vi "Check Trigger Conditions.vi"(7 "Force Trigger?":bool, 8 "error in (no error)":errorcluster, 9 "Waveform Data":waveform(sgl)[](array[waveform]), 10 "Acquisition and Logging Configuration":T1={"Data Rate"=1, "Samples per Read"=0, "Number of Reads to Save"=0, "Data File Name"="", "TDMS Properties"=[], "Number of Channels"=4, "Channel Scale Array"=[0.0, 0.0, 0.0, 0.0, 1.0, 1.0, 1.0, 1.0, 1.0, 1.0, 1.0, 1.0, 1.0, 1.0, 1.0, 1.0], "Channel Names"=[], "Trigger - RMS Value"=0.0, "Trigger - Channel"=0, "Trigger - Time (Minute)"=0, "Frequency "=0, "Amplitude (0~10)"=0.0} {"Amplitude (0~10)" min=-10.0 max=10.0; "Data Rate" items=["50.000 kS/s (NI 9239)"=1, "25.000 kS/s (NI 9239)"=2, "16.667 kS/s (NI 9239)"=3, "12.500 kS/s (NI 9239)"=4, "10.000 kS/s (NI 9239)"=5, "8.333 kS/s (NI 9239)"=6, "7.143 kS/s (NI 9239)"=7, "6.250 kS/s (NI 9239)"=8, "5.556 kS/s (NI 9239)"=9, "5.000 kS/s (NI 9239)"=10, "4.545 kS/s (NI 9239)"=11, "4.167 kS/s (NI 9239)"=12, "3.846 kS/s (NI 9239)"=13, "3.571 kS/s (NI 9239)"=14, "3.333 kS/s (NI 9239)"=15, "3.125 kS/s (NI 9239)"=16, "2.941 kS/s (NI 9239)"=17, "2.778 kS/s (NI 9239)"=18, "2.632 kS/s (NI 9239)"=19, "2.500 kS/s (NI 9239)"=20, "2.381 kS/s (NI 9239)"=21, "2.273 kS/s (NI 9239)"=22, "2.174 kS/s (NI 9239)"=23, "2.083 kS/s (NI 9239)"=24, "2.000 kS/s (NI 9239)"=25, "1.923 kS/s (NI 9239)"=26, "1.852 kS/s (NI 9239)"=27, "1.786 kS/s (NI 9239)"=28, "1.724 kS/s (NI 9239)"=29, "1.667 kS/s (NI 9239)"=30, "1.613 kS/s (NI 9239)"=31]}) -> (0 "error out":errorcluster, 3 "Trigger Condition Met?":bool)   [LabVIEW 2016]
uses:
  controls/Acquisition and Logging Configuration.ctl
  <vilib>/LabVIEW Targets/FPGA/cRIO/shared/nicrio_ModuleControls/nicrio_cRIO-9239_DataRatesRing.ctl
  controls/TDMS Properties.ctl
  <vilib>/Analysis/5stat.llb/RMS (DBL).vi
  <vilib>/Analysis/NI_AALPro.lvlib
panel:
  # "Verifica condições para início da aquisição, são elas:\n• Caso trigger seja forçado pela usuário\n• Caso o contador chegue no múltiplo correspondente ao Trigger - Time(Minute)\n• Caso o valor da forma de onda no canal escolhido seja alcançado\n• No caso do Trigger Minute = 0, dentro do arquivo de configuração, \nfoi convencionado que esse trigger sempre estará acionado para que aquisição nunca termine.\nEssa funcionalidade está documentada no diagrama de blocos."
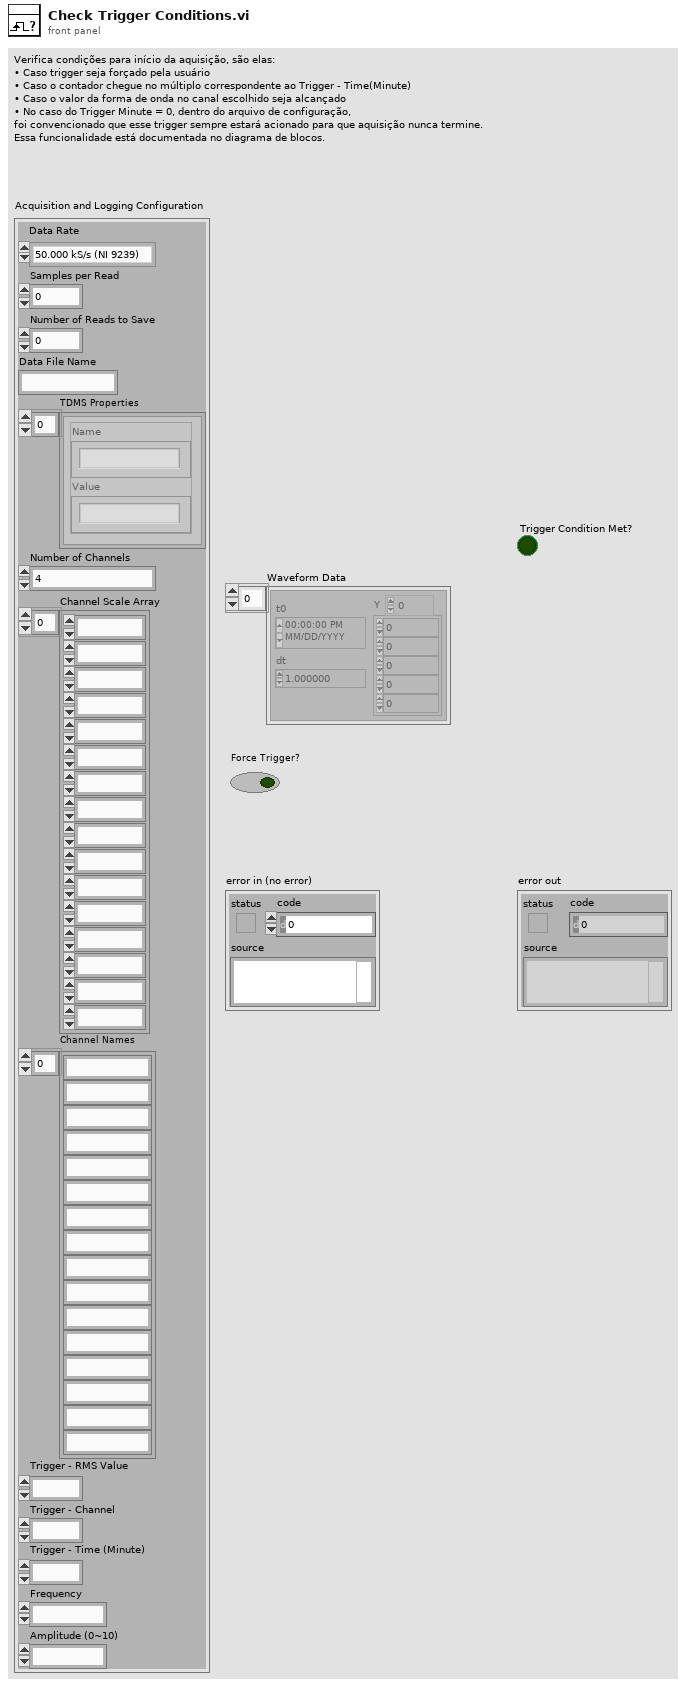
[diagram p1: front panel]
types:
  T1 = typedef "Acquisition and Logging Configuration.ctl" = cluster{"Data Rate":T2, "Samples per Read":i32, "Number of Reads to Save":i32, "Data File Name":string, "TDMS Properties":T3[], "Number of Channels":i32, "Channel Scale Array":fxp<+,24,12>[], "Channel Names":string[], "Trigger - RMS Value":dbl, "Trigger - Channel":i32, "Trigger - Time (Minute)":i32, "Frequency ":i32, "Amplitude (0~10)":dbl}
  T2 = typedef "nicrio_cRIO-9239_DataRatesRing.ctl" = u8
  T3 = typedef "TDMS Properties.ctl" = cluster{"Name":string, "Value":string}
  T4 = typedef "LVDateTimeRec.ctl" = cluster{"fractional second":dbl, "second":i32, "minute":i32, "hour":i32, "day of month":i32, "month":i32, "year":i32, "day of week":i32, "day of year":i32, "DST":i32}
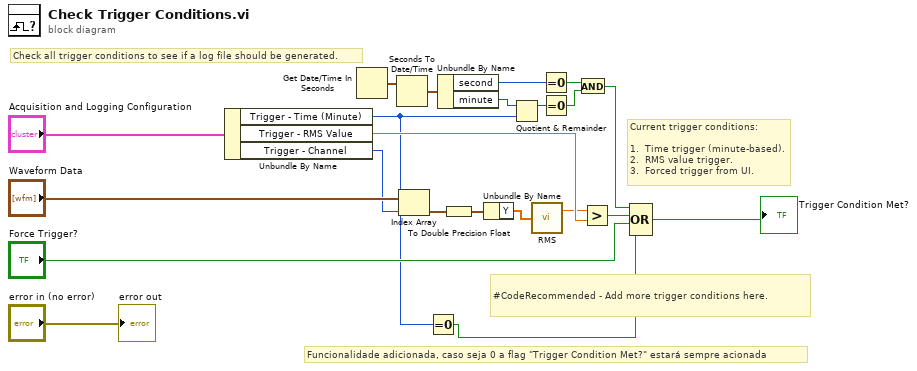
[diagram p0: block diagram]
diagram:
  # "Funcionalidade adicionada, caso seja 0 a flag \"Trigger Condition Met?\" estará sempre acionada"
  # "Check all trigger conditions to see if a log file should be generated."
  # "Current trigger conditions:\n\n1.  Time trigger (minute-based).\n2.  RMS value trigger.\n3.  Forced trigger from UI."
  # "#CodeRecommended - Add more trigger conditions here."
  n1 = Unbundle By Name("Acquisition and Logging Configuration") -> ("Trigger - Time (Minute)"=w3:i32, "Trigger - RMS Value"=w19:dbl, "Trigger - Channel"=w18:i32)
  n2 = Get Date/Time In Seconds() -> (seconds since 1Jan1904=w9:timestamp)
  n3 = Seconds To Date/Time(time stamp (now)=w9) -> (date time rec=w14:T4)  [unwired: 1 out]
  n4 = Index Array(array="Waveform Data", index=w18) -> (element=w17:waveform(sgl))
  n5 = Equal To 0?(x=w3) -> (x = 0?=w1:bool)
  n6 = Unbundle By Name(w14) -> ("second"=w2:i32, "minute"=w13:i32)
  n7 = To Double Precision Float(number=w17) -> (double precision float=w16:waveform(dbl))
  n8 = Unbundle By Name(w16) -> ("Y"=w5:dbl[])
  n9 = Quotient & Remainder(x=w13, y=w3) -> (x-y*floor(x/y)=w12:i32)  [unwired: 1 out]
  n10 = call-poly <vilib>:"RMS.vi"("X"=w5) -> ("rms value"=w4:dbl)  [unwired: 1 out]
  n11 = Equal To 0?(x=w2) -> (x = 0?=w11:bool)
  n12 = Equal To 0?(x=w12) -> (x = 0?=w10:bool)
  n13 = And(x=w11, y=w10) -> (x .and. y?=w7:bool)
  n14 = Greater?(x=w4, y=w19) -> (0:w15:bool)
  n15 = Compound Arithmetic op=OR(w7, w15, "Force Trigger?", w1) -> (→"Trigger Condition Met?":bool)
  "error out" <- "error in (no error)"
